vi "DC Supply Control.vi"(8 "error in":errorcluster, 10 "VISA res in":refnum<visa-resource-name>, 11 "HTS Results in":refnum<class "HTS Results.lvclass">) -> (0 "error out":errorcluster, 1 "Supp I":dbl, 2 "VISA res out":refnum<visa-resource-name>, 3 "HTS Results out":refnum<class "HTS Results.lvclass">)   [LabVIEW 2019, in "Results.lvlib" / "HTS Results.lvclass"]
uses:
  HTS Results.lvclass
  HTS Results.lvclass/HTS Results.ctl
  DAC/HTS/DC Supply/DAC DC Supply.lvclass
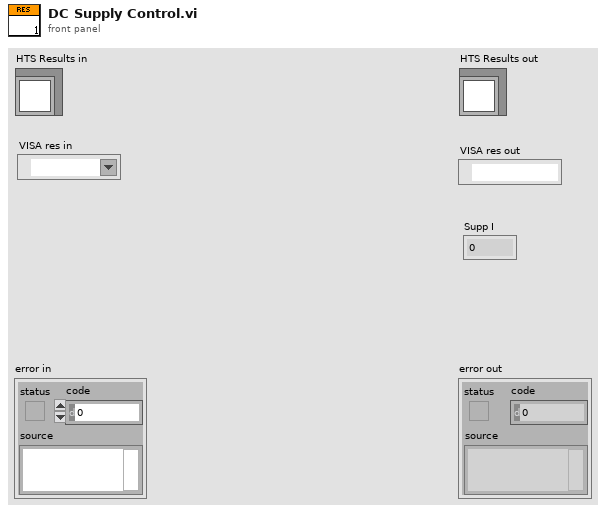
[diagram p1: front panel]
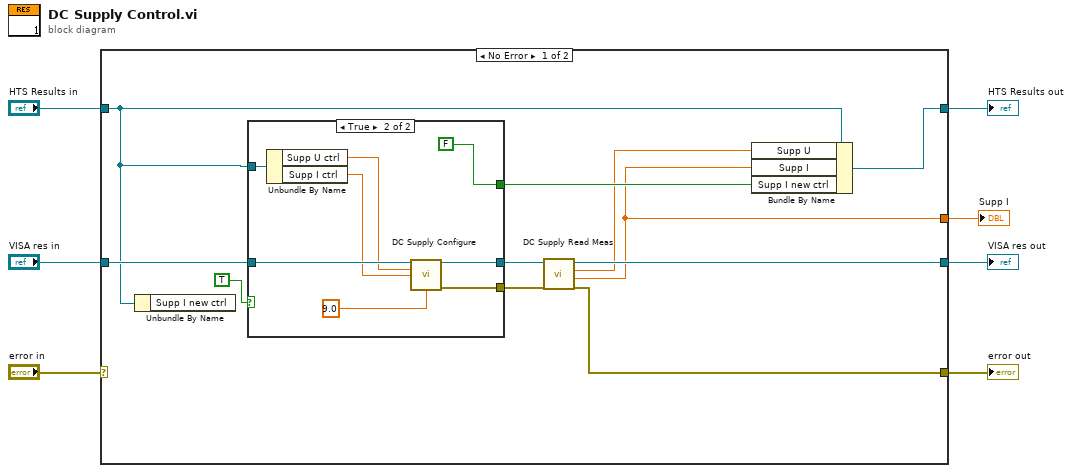
[diagram p0: block diagram]
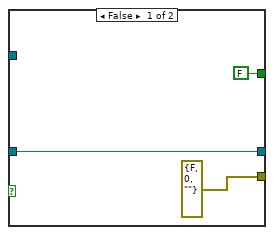
[diagram p2: hidden frame]
diagram:
  n1 = case shown="No Error" "error in" {
    selector: "error in" -> [_ w32]
    tunnel: [w10 w32] -> w6
    tunnel: [w18 w31] -> w4
    tunnel: "HTS Results in" -> [w16 w31]
    tunnel: "VISA res in" -> [w17 w30]
    tunnel: [w12 w30] -> w2
    tunnel: [w8 _] -> w1
    frame No Error {
      n2 = Unbundle By Name(w16) -> ()  [unwired: 1 out]
      n3 = case shown="True" TRUE {
        tunnel: w17 -> [w21 w27]
        tunnel: w16 -> [_ w29]
        tunnel: [w21 w26] -> w13
        tunnel: [errorcluster {"status"=FALSE, "code"=0, "source"=""} ("error out") w25] -> w11
        tunnel: [FALSE ("Supp I new ctrl") FALSE ("Supp I new ctrl")] -> w15
        frame False {
        }
        frame True {
          n4 = Unbundle By Name(w29) -> ("Supp U ctrl"=w23:dbl, "Supp I ctrl"=w24:dbl)
          n5 = call "DC Supply Configure.vi"("VISA resource name"=w27, "Voltage(0 Volts)"=w23, "Current(0 Amps)"=w24, "Overvoltage prot value"=9.0 ("Overvoltage prot value(50 Volts)")) -> ("VISA resource name out"=w26:refnum<visa-resource-name>, "error out"=w25:errorcluster)  [unwired: 10 in]
        }
      }
      n6 = call "DC Supply Read Meas.vi"("error in"=w11, "VISA resource name"=w13) -> ("error out"=w10:errorcluster, "Current (Amps)"=w8:dbl, "Voltage (Volts)"=w9:dbl, "VISA resource name out"=w12:refnum<visa-resource-name>)  [unwired: 6 in]
      n7 = Bundle By Name(cluster=w16, "Supp U"=w9, "Supp I"=w8, "Supp I new ctrl"=w15) -> (w18:refnum<class "HTS Results.lvclass">)
    }
    frame Error {
    }
  }
  "error out" <- w6
  "HTS Results out" <- w4
  "VISA res out" <- w2
  "Supp I" <- w1
